vi "Make String Safe.vi"(8 "Error in":errorcluster caption="Error in (no error)", 11 "Raw String":string) -> (0 "Error out":errorcluster, 3 "String out":string)   [LabVIEW 2023, in "Confluence Formatting.lvlib"]
uses:
  Confluence Formatting.lvlib
  <userlib>/_PetranWay/LabVIEW Confluence API/Source/PetranWay_Confluence API.lvlib
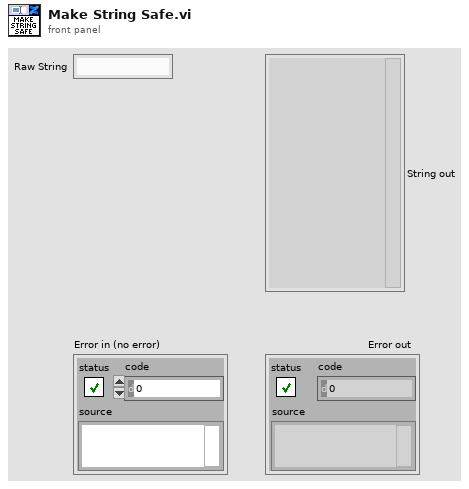
[diagram p1: front panel]
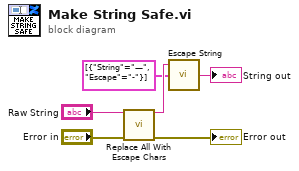
[diagram p0: block diagram]
diagram:
  n1 = call <userlib>:"Replace All With Escape Chars.vi"("Raw String"="Raw String", "error in (no error)"="Error in") -> ("With Substitued Escape Characters"=w6:string, "error out"=→"Error out":errorcluster)  [unwired: 12 in]
  n2 = call <vilib>:"Escape String.vi"("Escapes"=cluster{"String":string, "Escape":string}[] [{"String"="—", "Escape"="-"}], "String in"=w6) -> ("String out"=→"String out":string)  [unwired: 1 in]
